vi "AD9910.vi"() -> ()   [LabVIEW 2018]
panel:
  in  "Name":string
  out "SN":u16 format="%04x"
  in  "Save Button":bool
  out "Save Config":path
  in  "Open Config":path
  out "Error":errorcluster
  in  "Stop":bool
  in  "Enable Sine Out":bool
  in  "Enable Profile ASF":bool
  in  "Profiles":enum32{"Single Tone", "RAM"}(tab)
  in  "Single Tone 0":T1 {"Phase" step=0.1 format="%.5f"; "Power" min=0.0 max=0.0009998779334127903 step=5e-05 format="%.9f"; "Frequency" min=0.0 max=500000000.0 format="%.7f"}
  in  "Single Tone 1":T1 {"Phase" step=0.1 format="%.5f"; "Power" min=0.0 max=0.0009998779334127903 step=5e-05 format="%.9f"; "Frequency" min=0.0 max=500000000.0 format="%.7f"}
  in  "Single Tone 2":T1 {"Phase" step=0.1 format="%.5f"; "Power" min=0.0 max=0.0009998779334127903 step=5e-05 format="%.9f"; "Frequency" min=0.0 max=500000000.0 format="%.7f"}
  in  "Single Tone 3":T1 {"Phase" step=0.1 format="%.5f"; "Power" min=0.0 max=0.0009998779334127903 step=5e-05 format="%.9f"; "Frequency" min=0.0 max=500000000.0 format="%.7f"}
  in  "Single Tone 4":T1 {"Phase" step=0.1 format="%.5f"; "Power" min=0.0 max=0.0009998779334127903 step=5e-05 format="%.9f"; "Frequency" min=0.0 max=500000000.0 format="%.7f"}
  in  "Single Tone 5":T1 {"Phase" step=0.1 format="%.5f"; "Power" min=0.0 max=0.0009998779334127903 step=5e-05 format="%.9f"; "Frequency" min=0.0 max=500000000.0 format="%.7f"}
  in  "Single Tone 6":T1 {"Phase" step=0.1 format="%.5f"; "Power" min=0.0 max=0.0009998779334127903 step=5e-05 format="%.9f"; "Frequency" min=0.0 max=500000000.0 format="%.7f"}
  in  "Single Tone 7":T1 {"Phase" step=0.1 format="%.5f"; "Power" min=0.0 max=0.0009998779334127903 step=5e-05 format="%.9f"; "Frequency" min=0.0 max=500000000.0 format="%.7f"}
  in  "Activate":T2(radio)
  in  "ADIClockEval":u16(ring) items=["not 780 X- Local Detection_is raman S&H", "780_X+_Local_Detection", "1529 Shielding", "420 S&H", "808 SLM", "420 Slow Feedback"]
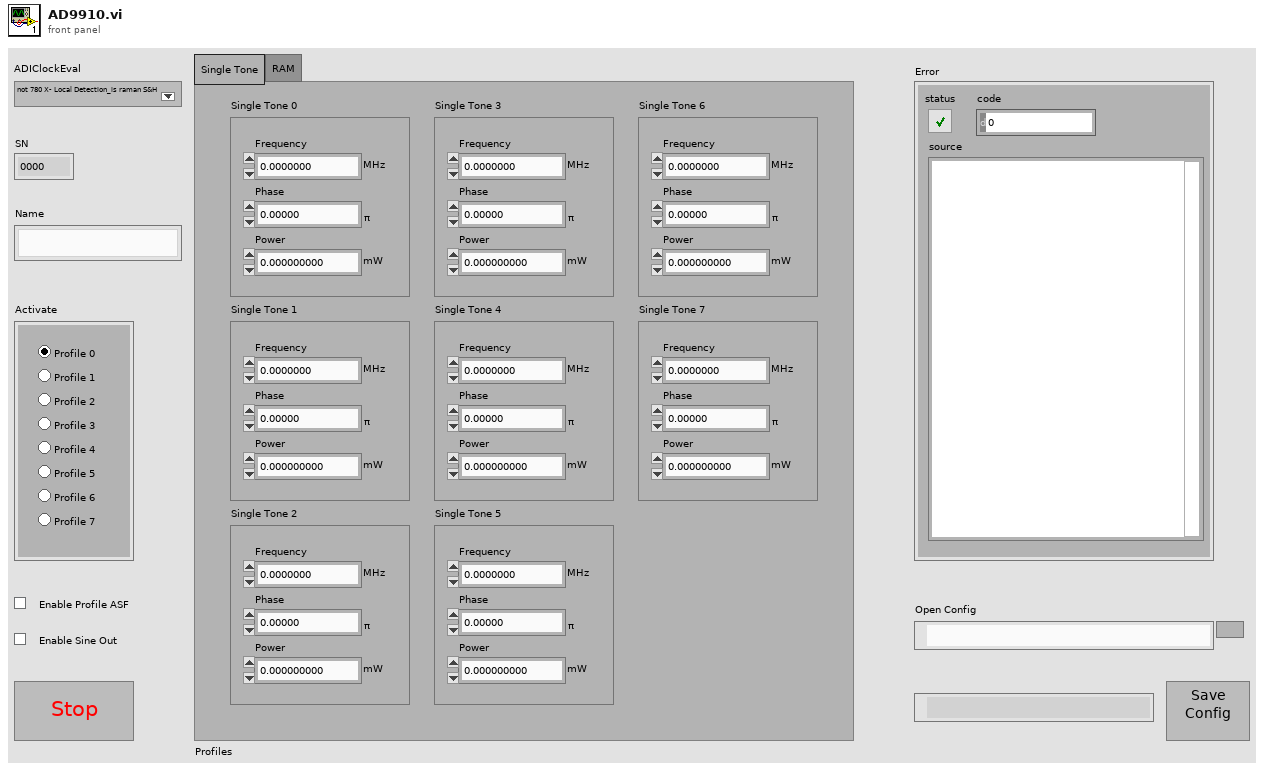
[diagram p1: front panel]
types:
  T1 = cluster{"Frequency":dbl[unit], "Phase":dbl, "Power":dbl[unit]}
  T2 = enum32{"单选选项0", "单选选项1", "单选选项2", "单选选项3", "单选选项4", "单选选项5", "单选选项6", "单选选项7"}
  T3 = cluster{"[0]":enum8{"Enabled", "Disabled", "Disabled and Grayed Out"}, "[1]":enum8{"Enabled", "Disabled", "Disabled and Grayed Out"}, "[2]":enum8{"Enabled", "Disabled", "Disabled and Grayed Out"}, "[3]":enum8{"Enabled", "Disabled", "Disabled and Grayed Out"}, "[4]":enum8{"Enabled", "Disabled", "Disabled and Grayed Out"}, "[5]":enum8{"Enabled", "Disabled", "Disabled and Grayed Out"}, "[6]":enum8{"Enabled", "Disabled", "Disabled and Grayed Out"}, "[7]":enum8{"Enabled", "Disabled", "Disabled and Grayed Out"}}
  T4 = cluster{"Single Tone 0":cluster{"Frequency":dbl[unit], "Phase":dbl, "Power":dbl[unit]}, "Single Tone 1":cluster{"Frequency":dbl[unit], "Phase":dbl, "Power":dbl[unit]}, "Single Tone 2":cluster{"Frequency":dbl[unit], "Phase":dbl, "Power":dbl[unit]}, "Single Tone 3":cluster{"Frequency":dbl[unit], "Phase":dbl, "Power":dbl[unit]}, "Single Tone 4":cluster{"Frequency":dbl[unit], "Phase":dbl, "Power":dbl[unit]}, "Single Tone 5":cluster{"Frequency":dbl[unit], "Phase":dbl, "Power":dbl[unit]}, "Single Tone 6":cluster{"Frequency":dbl[unit], "Phase":dbl, "Power":dbl[unit]}, "Single Tone 7":cluster{"Frequency":dbl[unit], "Phase":dbl, "Power":dbl[unit]}}
  T5 = enum8{"Enabled", "Disabled", "Disabled and Grayed Out"}
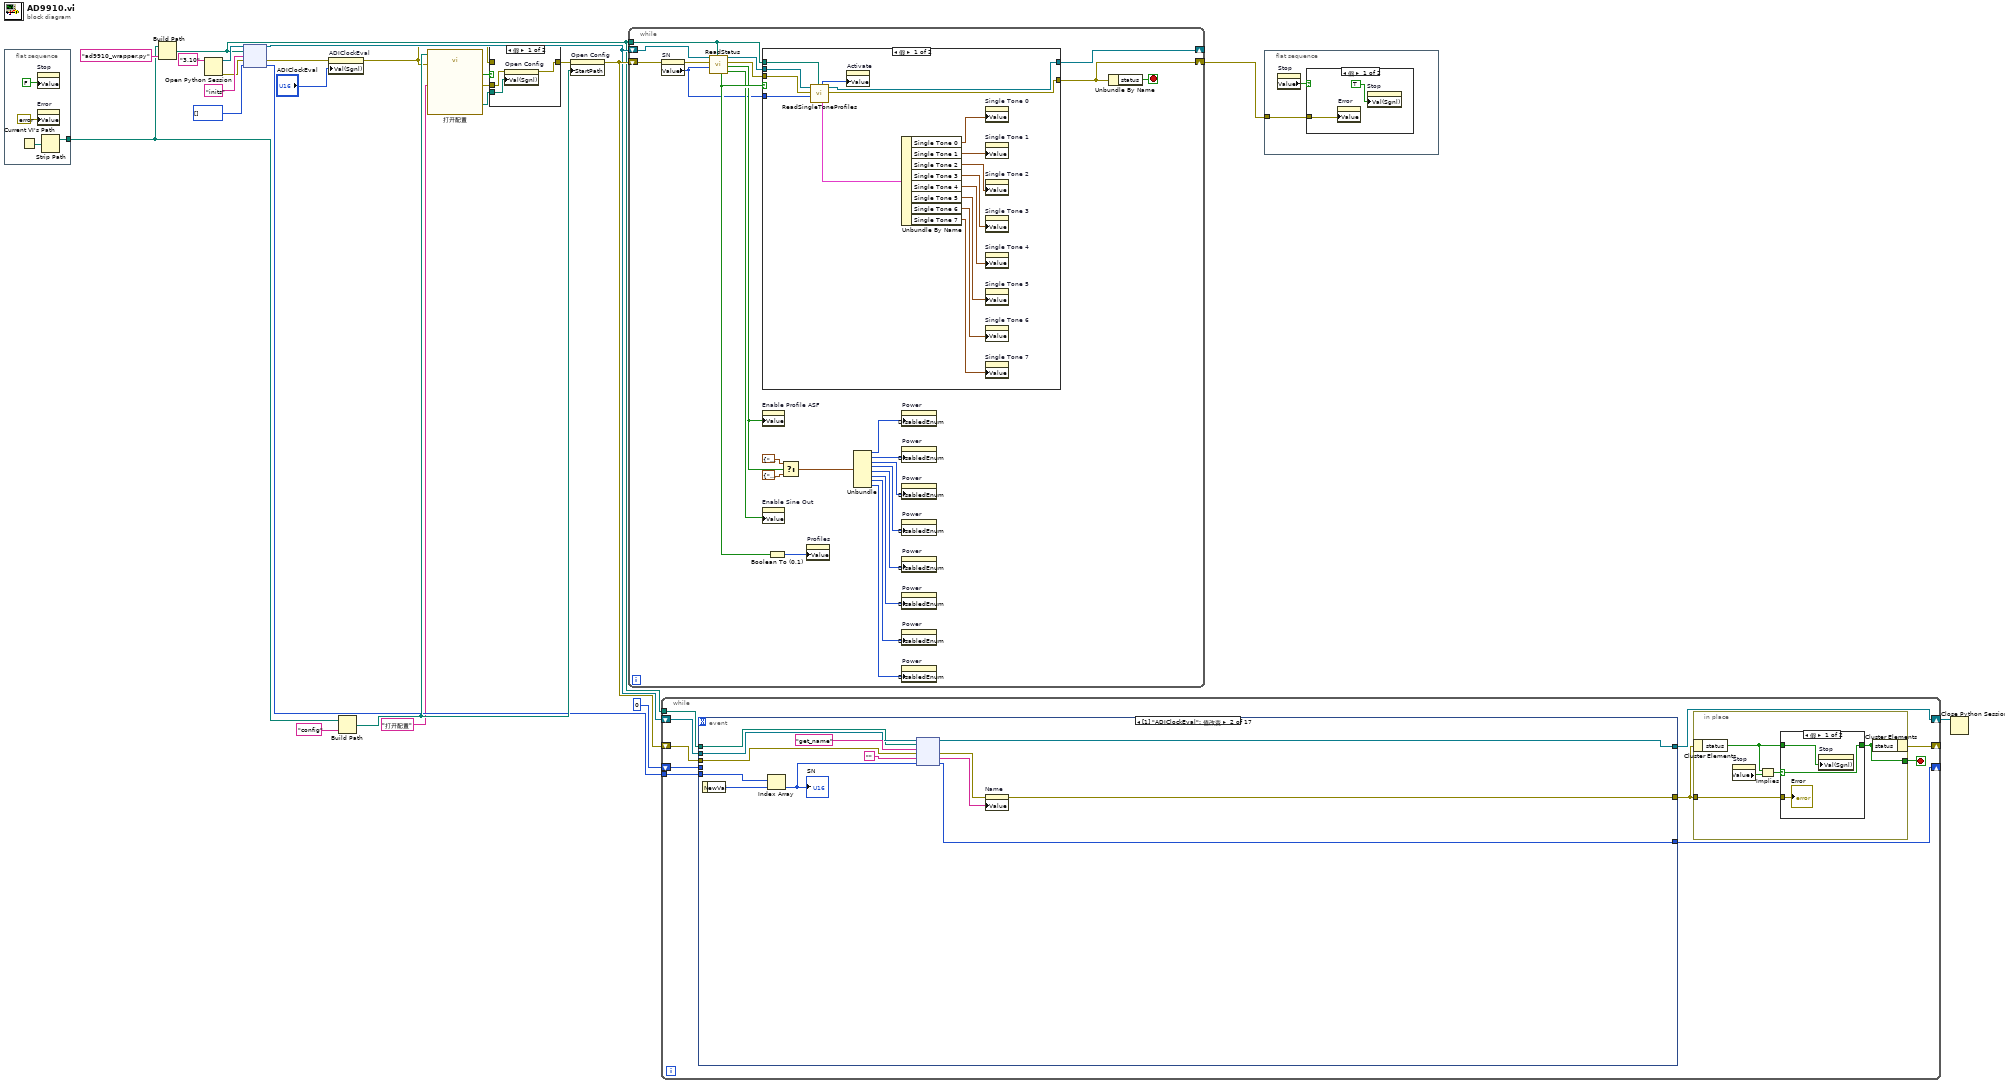
[diagram p0: block diagram]
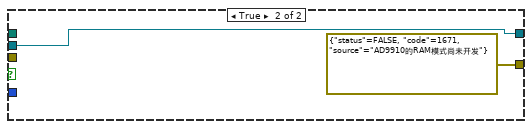
[diagram p4: hidden frame]
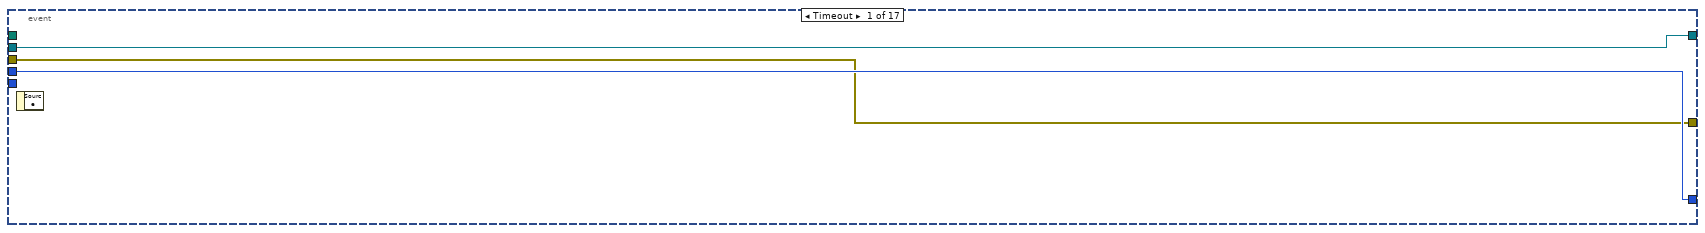
[diagram p6: hidden frame]
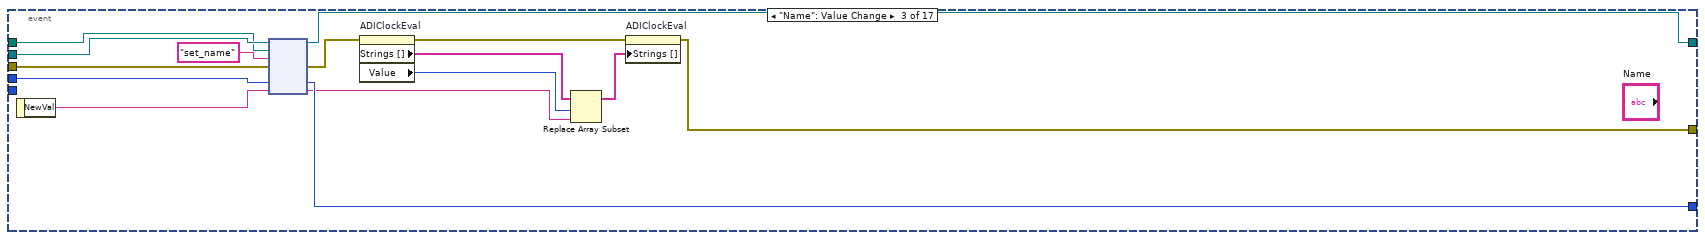
[diagram p7: hidden frame]
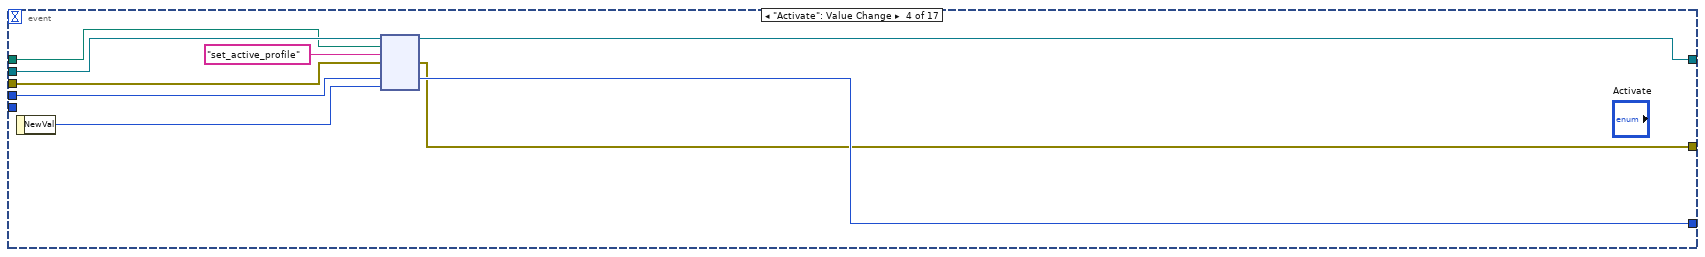
[diagram p8: hidden frame]
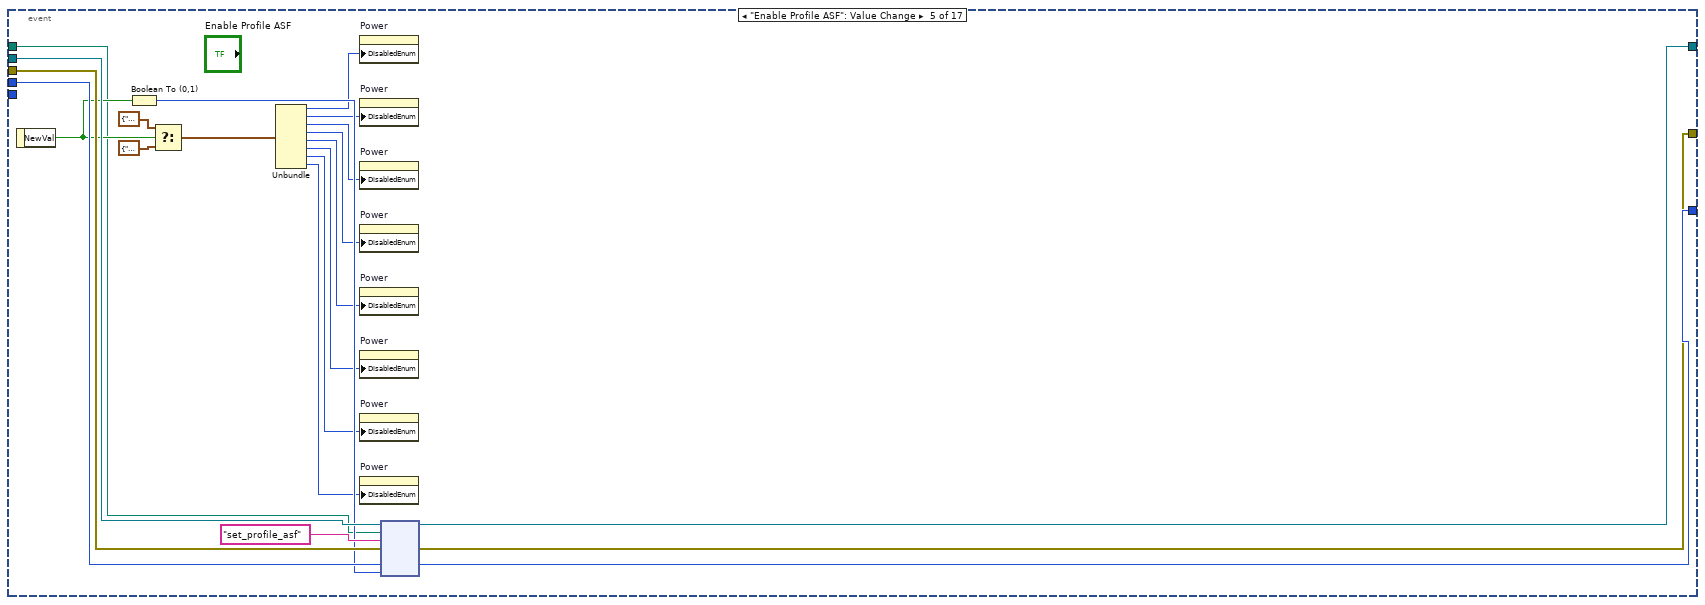
[diagram p9: hidden frame]
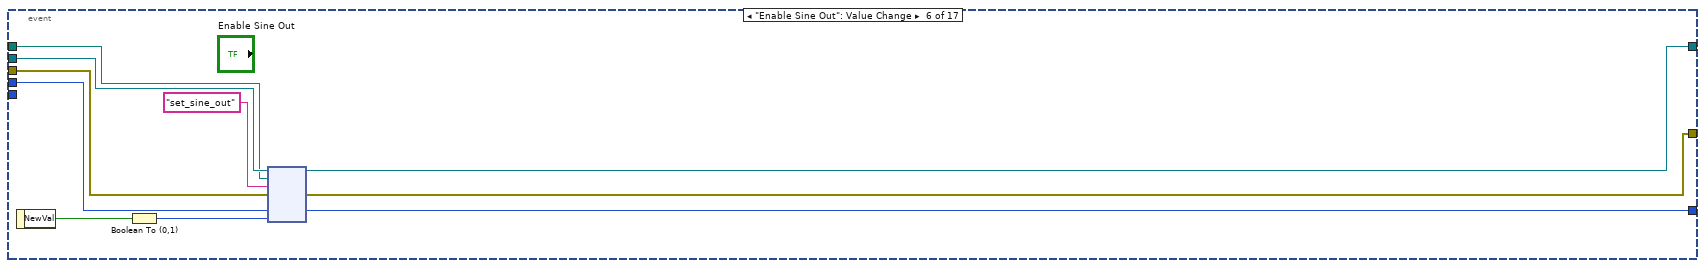
[diagram p10: hidden frame]
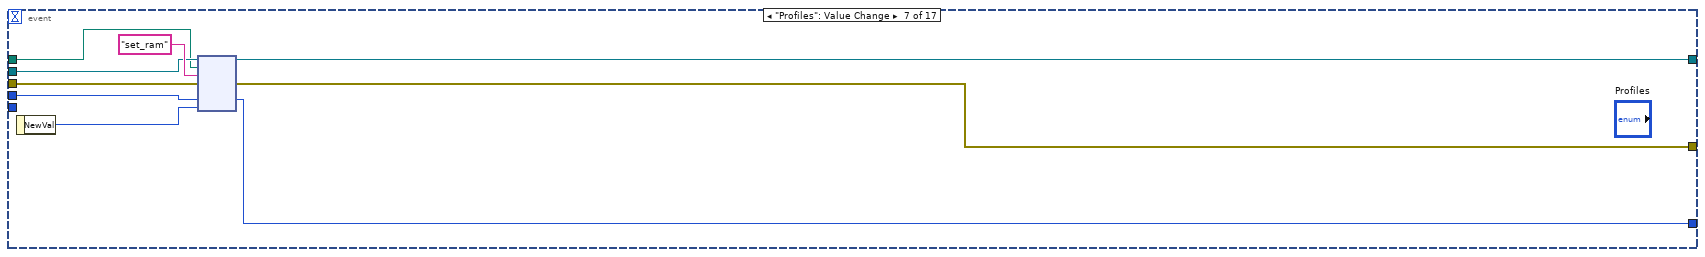
[diagram p11: hidden frame]
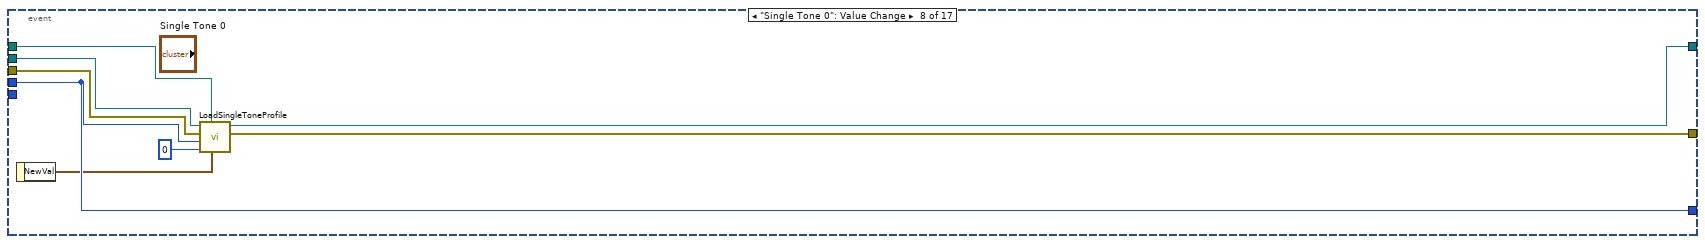
[diagram p12: hidden frame]
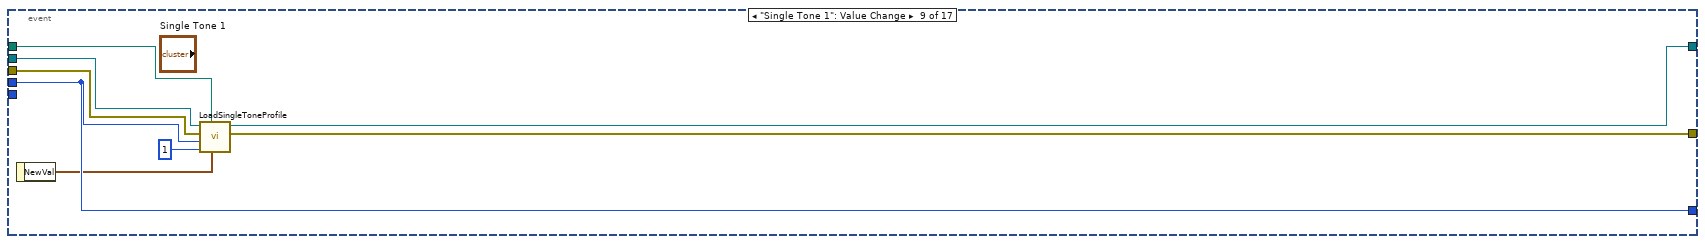
[diagram p13: hidden frame]
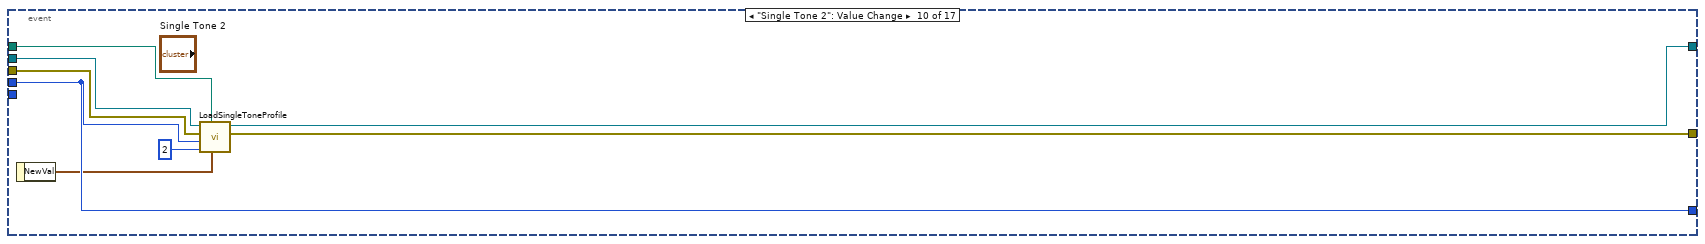
[diagram p14: hidden frame]
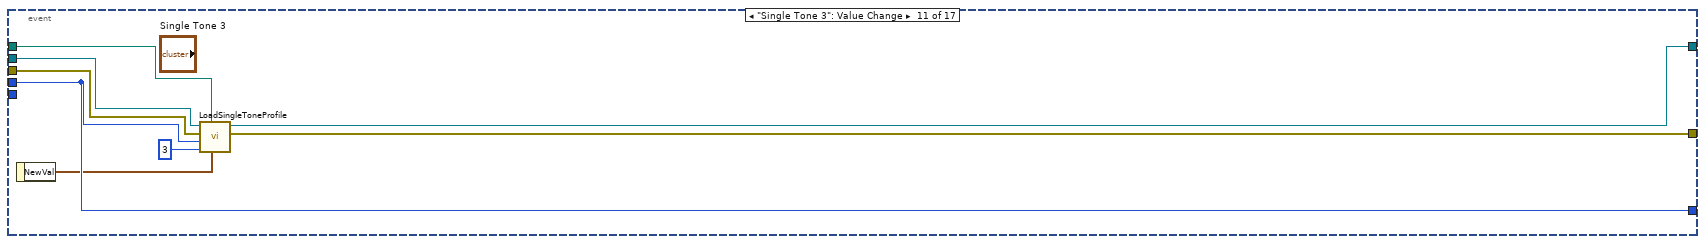
[diagram p15: hidden frame]
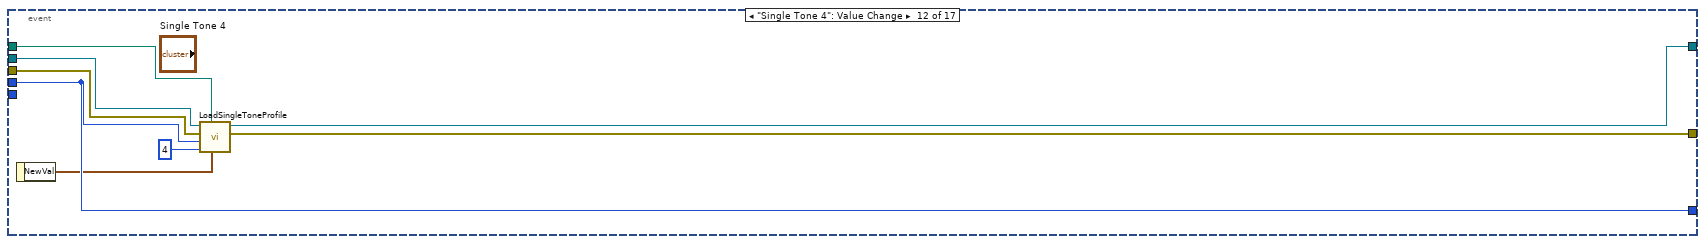
[diagram p16: hidden frame]
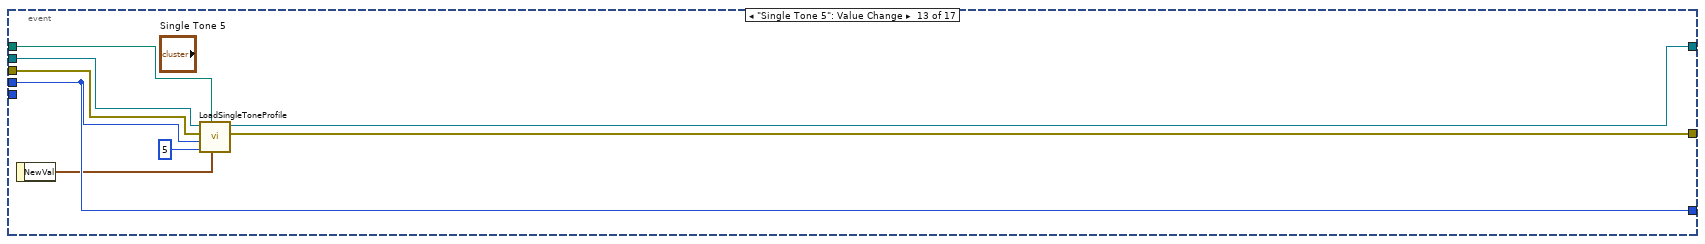
[diagram p17: hidden frame]
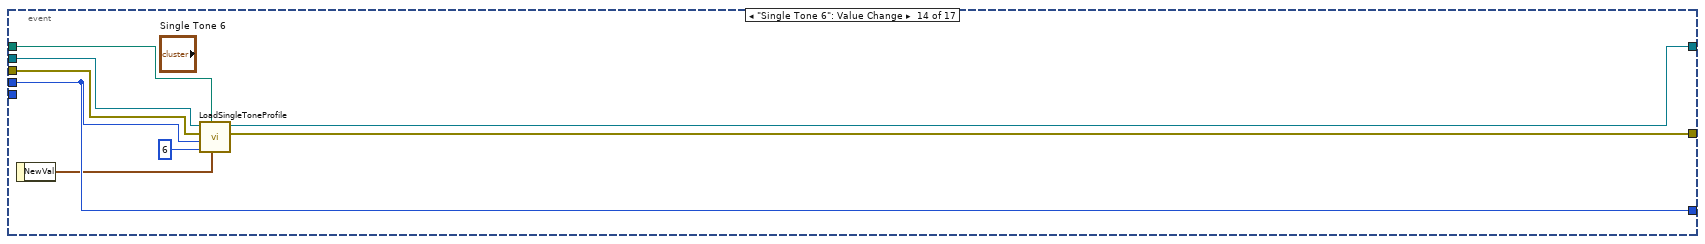
[diagram p18: hidden frame]
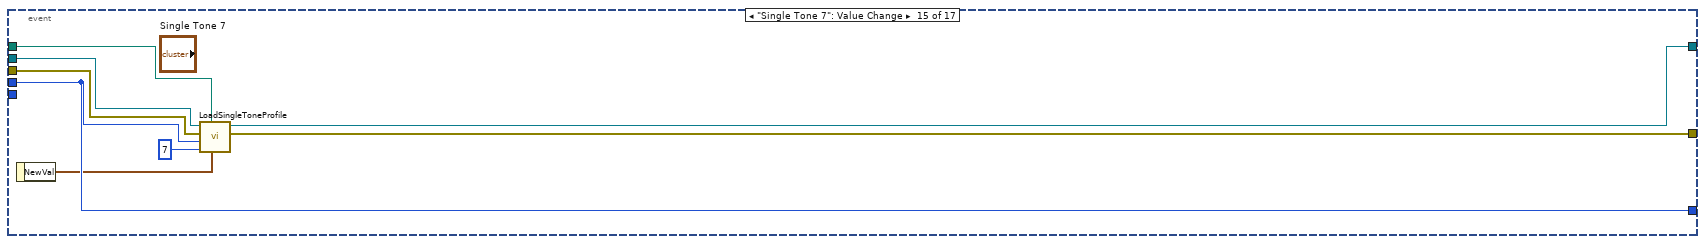
[diagram p19: hidden frame]
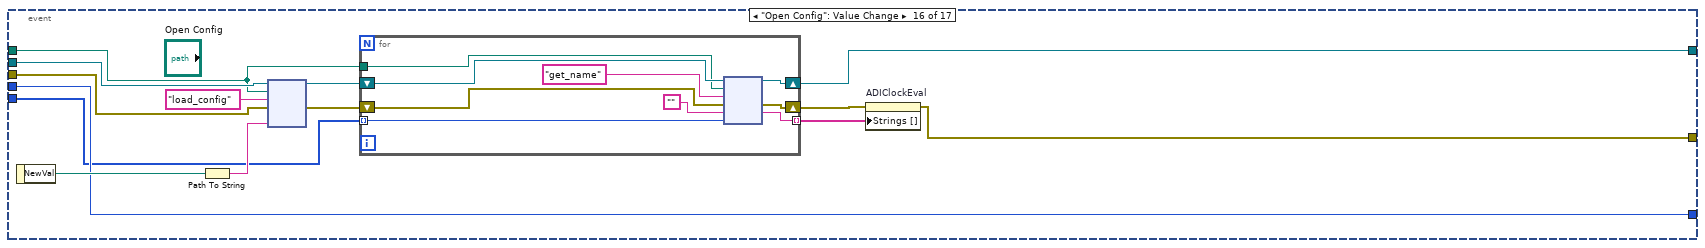
[diagram p20: hidden frame]
diagram:
  n1 = flat-sequence {
    tunnel: [w27] -> w16
    frame #0 {
      n2 = Current VI's Path() -> (path=w28:path)
      n3 = property on="Stop" class="Bool (严格)"("Value"=FALSE ("Stop")) -> ()  [unwired: 2 in, 2 out]
      n4 = property on="Error" class="Clust (严格)"("Value"=errorcluster {"status"=FALSE, "code"=0, "source"=""} ("Error")) -> ()  [unwired: 2 in, 2 out]
      n5 = Strip Path(path=w28) -> (stripped path=w27:path)  [unwired: 1 out]
    }
  }
  n6 = Build Path(base path=w16, name or relative path="ad9910_wrapper.py") -> (appended path=w10:path)
  n7 = Open Python Session(python version="3.10" ("Python版本")) -> (session out=w23:refnum<k35>, error out=w21:errorcluster)  [unwired: 2 in]
  n8 = node ("Python节点")(w23, w10, "inits", w21, u16[] []) -> (w11:refnum<k35>, w3:errorcluster, w9:u16[])  [unwired: 2 out]
  n9 = property on="ADIClockEval" class="Ring (严格)"(error in=w3, "Val(Sgnl)"="ADIClockEval") -> (error out=w2:errorcluster)  [unwired: 1 in, 1 out]
  n10 = Build Path(base path=w16, name or relative path="config") -> (appended path=w15:path)
  n11 = call "打开配置"("start path"=w15, "prompt"="打开配置" ("default name"), "error in"=w2) -> ("selected path"=w6:path, "cancelled"=w7:bool, "error out"=w5:errorcluster)  [unwired: 9 in, 1 out]
  n12 = case shown="假" w7 {
    tunnel: w6 -> [w31 _]
    tunnel: w5 -> [w30 _]
    tunnel: [w29 w32] -> w14
    tunnel: w2 -> [_ w32]
    frame False {
      n13 = property on="Open Config" class="Path"(error in=w30, "Val(Sgnl)"=w31) -> (error out=w29:errorcluster)  [unwired: 1 in, 1 out]
    }
    frame True {
    }
  }
  n14 = property on="Open Config" class="Path"(error in=w14, "StartPath"=w15) -> (error out=w13:errorcluster)  [unwired: 1 in, 1 out]
  n15 = while {
    shift-right: [w36] -> _
    shift-left: w11 -> [w42]
    shift-right: [w37] -> w18
    shift-left: w13 -> [w35]
    tunnel: w10 -> [w40]
    stop <- w41 stop-if-true
    n16 = property on="SN" class="DigNum (严格)"(error in=w35) -> (error out=w34:errorcluster, "Value"=w33:u16)  [unwired: 1 in, 1 out]
    n17 = call "ReadStatus.vi"("模块路径"=w40, "sn"=w33, "错误输入（无错误）"=w34, "会话句柄输入"=w42) -> ("Enable Sine Out"=w47:bool, "Enable Profile ASF"=w45:bool, "错误输出"=w39:errorcluster, "会话句柄输出"=w38:refnum<k35>, "Enable RAM"=w49:bool)  [unwired: 3 in]
    n18 = case shown="假" w49 {
      tunnel: w38 -> [w73 w74]
      tunnel: w39 -> [w72 _]
      tunnel: w33 -> [w71 _]
      tunnel: [w70 errorcluster {"status"=FALSE, "code"=1671, "source"="AD9910的RAM模式尚未开发"} ("错误输出")] -> w37
      tunnel: [w69 w74] -> w36
      tunnel: w40 -> [w58 _]
      frame False {
        n19 = call "ReadSingleToneProfiles.vi"("模块路径"=w58, "sn"=w71, "错误输入（无错误）"=w72, "会话句柄输入"=w73) -> ("错误输出"=w70:errorcluster, "会话句柄输出"=w69:refnum<k35>, "Single Tone Profiles"=w68:T4, "Activate"=w67:T2)  [unwired: 4 in]
        n20 = property on="Activate" class="RadioBtnsControl (严格)"("Value"=w67) -> ()  [unwired: 2 in, 2 out]
        n21 = Unbundle By Name(w68) -> ("Single Tone 0"=w66:T1, "Single Tone 1"=w65:T1, "Single Tone 2"=w64:T1, "Single Tone 3"=w63:T1, "Single Tone 4"=w62:T1, "Single Tone 5"=w61:T1, "Single Tone 6"=w60:T1, "Single Tone 7"=w59:T1)
        n22 = property on="Single Tone 0" class="Clust (严格)"("Value"=w66) -> ()  [unwired: 2 in, 2 out]
        n23 = property on="Single Tone 1" class="Clust (严格)"("Value"=w65) -> ()  [unwired: 2 in, 2 out]
        n24 = property on="Single Tone 2" class="Clust (严格)"("Value"=w64) -> ()  [unwired: 2 in, 2 out]
        n25 = property on="Single Tone 3" class="Clust (严格)"("Value"=w63) -> ()  [unwired: 2 in, 2 out]
        n26 = property on="Single Tone 4" class="Clust (严格)"("Value"=w62) -> ()  [unwired: 2 in, 2 out]
        n27 = property on="Single Tone 5" class="Clust (严格)"("Value"=w61) -> ()  [unwired: 2 in, 2 out]
        n28 = property on="Single Tone 6" class="Clust (严格)"("Value"=w60) -> ()  [unwired: 2 in, 2 out]
        n29 = property on="Single Tone 7" class="Clust (严格)"("Value"=w59) -> ()  [unwired: 2 in, 2 out]
      }
      frame True {
      }
    }
    n30 = property on="Enable Profile ASF" class="Bool (严格)"("Value"=w45) -> ()  [unwired: 2 in, 2 out]
    n31 = property on="Enable Sine Out" class="Bool (严格)"("Value"=w47) -> ()  [unwired: 2 in, 2 out]
    n32 = Boolean To (0,1)(Boolean=w49) -> (0, 1=w48:i16)
    n33 = Select(t=T3 {"[0]"=enum."Enabled", "[1]"=enum."Enabled", "[2]"=enum."Enabled", "[3]"=enum."Enabled", "[4]"=enum."Enabled", "[5]"=enum."Enabled", "[6]"=enum."Enabled", "[7]"=enum."Enabled"} ("簇"), s=w45, f=T3 {"[0]"=enum."Disabled and Grayed Out", "[1]"=enum."Disabled and Grayed Out", "[2]"=enum."Disabled and Grayed Out", "[3]"=enum."Disabled and Grayed Out", "[4]"=enum."Disabled and Grayed Out", "[5]"=enum."Disabled and Grayed Out", "[6]"=enum."Disabled and Grayed Out", "[7]"=enum."Disabled and Grayed Out"} ("簇")) -> (s? t:f=w46:T3)
    n34 = property on="Profiles" class="TabCtl (严格)"("Value"=w48) -> ()  [unwired: 2 in, 2 out]
    n35 = Unbundle(w46) -> ("[0]"=w50:T5, "[1]"=w51:T5, "[2]"=w52:T5, "[3]"=w53:T5, "[4]"=w54:T5, "[5]"=w55:T5, "[6]"=w56:T5, "[7]"=w57:T5)
    n36 = property on="Power" class="DigNum (严格)"("DisabledEnum"=w50) -> ()  [unwired: 2 in, 2 out]
    n37 = property on="Power" class="DigNum (严格)"("DisabledEnum"=w51) -> ()  [unwired: 2 in, 2 out]
    n38 = property on="Power" class="DigNum (严格)"("DisabledEnum"=w52) -> ()  [unwired: 2 in, 2 out]
    n39 = property on="Power" class="DigNum (严格)"("DisabledEnum"=w53) -> ()  [unwired: 2 in, 2 out]
    n40 = property on="Power" class="DigNum (严格)"("DisabledEnum"=w54) -> ()  [unwired: 2 in, 2 out]
    n41 = property on="Power" class="DigNum (严格)"("DisabledEnum"=w55) -> ()  [unwired: 2 in, 2 out]
    n42 = property on="Power" class="DigNum (严格)"("DisabledEnum"=w56) -> ()  [unwired: 2 in, 2 out]
    n43 = property on="Power" class="DigNum (严格)"("DisabledEnum"=w57) -> ()  [unwired: 2 in, 2 out]
    n44 = Unbundle By Name(w37) -> ("status"=w41:bool)
  }
  n45 = while {
    tunnel: w9 -> [w80]
    shift-right: [w82] -> _
    shift-left: u16 0 -> [w84]
    shift-right: [w78] -> _
    shift-left: w13 -> [w81]
    shift-right: [w83] -> w12
    shift-left: w11 -> [w85]
    tunnel: w10 -> [w79]
    stop <- w77 stop-if-true
    n46 = event shown="[1] \"ADIClockEval\": 值改变" {
      selector: _ -> [_ _ _ _ _ _ _ _ _ _ _ _ _ _ _ _ _]
      dyn-events: _ -> [_ _ _ _ _ _ _ _ _ _ _ _ _ _ _ _ _]
      timeout: _ -> [_ _ _ _ _ _ _ _ _ _ _ _ _ _ _ _ _]
      tunnel: w81 -> [w96 w98 w122 w133 w153 w163 w172 w181 w189 w197 w205 w213 w221 w229 w237 w248 w284]
      tunnel: w85 -> [w95 w104 w125 w134 w154 w164 w173 w182 w190 w198 w206 w214 w222 w230 w238 w249 w274]
      tunnel: w84 -> [w97 _ w121 w132 w152 w162 w171 w178 w186 w194 w202 w210 w218 w226 w234 w247 w268]
      tunnel: [w95 w103 w119 w129 w149 w158 w170 w177 w185 w193 w201 w209 w217 w225 w233 w243 w263] -> w83
      tunnel: [w97 w102 w118 w130 w150 w160 w168 w178 w186 w194 w202 w210 w218 w226 w234 w247 w268] -> w82
      tunnel: w80 -> [_ w109 _ _ _ _ _ _ _ _ _ _ _ _ _ w246 _]
      tunnel: w79 -> [_ w101 w124 w126 w135 w156 w166 w175 w183 w191 w199 w207 w215 w223 w231 w242 w262]
      tunnel: [w96 w100 w113 w128 w148 w159 w169 w179 w187 w195 w203 w211 w219 w227 w235 w240 w265] -> w76
      event Timeout {
        n47 = event-data() -> ()  [unwired: 1 in, 1 out]
      }
      event "ADIClockEval": Value Change {
        n48 = event-data() -> ("NewVal"=w110:u16)  [unwired: 1 in]
        n49 = Index Array(array=w109, index=w110) -> (element=w99:u16)
        "SN" <- w99
        n50 = node(w104, w101, "get_name", w98, "", w99) -> (w103:refnum<k35>, w108:errorcluster, w107:string, w102:u16)  [unwired: 2 out]
        n51 = property on="Name" class="Str"(error in=w108, "Value"=w107) -> (error out=w100:errorcluster)  [unwired: 1 in, 1 out]
      }
      event "Name": Value Change {
        n52 = event-data() -> ("NewVal"=w120:string)  [unwired: 1 in]
        n53 = node(w125, w124, "set_name", w122, w121, w120) -> (w119:refnum<k35>, w117:errorcluster, w118:u16, w114:string)  [unwired: 2 in, 2 out]
        n54 = property on="ADIClockEval" class="Ring (严格)"(error in=w117) -> (error out=w111:errorcluster, "Strings []"=w116:string[], "Value"=w115:u16)  [unwired: 1 in, 1 out]
        n55 = Replace Array Subset(array=w116, new element=w114, index=w115) -> (w112:string[])
        n56 = property on="ADIClockEval" class="Ring (严格)"(error in=w111, "Strings []"=w112) -> (error out=w113:errorcluster)  [unwired: 1 in, 1 out]
      }
      event "Activate": Value Change {
        n57 = event-data() -> ("NewVal"=w127:T2)  [unwired: 1 in]
        n58 = node(w134, w126, "set_active_profile", w133, w132, w127) -> (w129:refnum<k35>, w128:errorcluster, w130:u16)  [unwired: 3 in, 2 out]
      }
      event "Enable Profile ASF": Value Change {
        n59 = event-data() -> ("NewVal"=w136:bool)  [unwired: 1 in]
        n60 = Boolean To (0,1)(Boolean=w136) -> (0, 1=w151:i16)
        n61 = Select(t=T3 {"[0]"=enum."Enabled", "[1]"=enum."Enabled", "[2]"=enum."Enabled", "[3]"=enum."Enabled", "[4]"=enum."Enabled", "[5]"=enum."Enabled", "[6]"=enum."Enabled", "[7]"=enum."Enabled"} ("簇"), s=w136, f=T3 {"[0]"=enum."Disabled and Grayed Out", "[1]"=enum."Disabled and Grayed Out", "[2]"=enum."Disabled and Grayed Out", "[3]"=enum."Disabled and Grayed Out", "[4]"=enum."Disabled and Grayed Out", "[5]"=enum."Disabled and Grayed Out", "[6]"=enum."Disabled and Grayed Out", "[7]"=enum."Disabled and Grayed Out"} ("簇")) -> (s? t:f=w147:T3)
        n62 = Unbundle(w147) -> ("[0]"=w146:T5, "[1]"=w145:T5, "[2]"=w144:T5, "[3]"=w143:T5, "[4]"=w142:T5, "[5]"=w141:T5, "[6]"=w140:T5, "[7]"=w139:T5)
        n63 = property on="Power" class="DigNum (严格)"("DisabledEnum"=w146) -> ()  [unwired: 2 in, 2 out]
        n64 = property on="Power" class="DigNum (严格)"("DisabledEnum"=w145) -> ()  [unwired: 2 in, 2 out]
        n65 = property on="Power" class="DigNum (严格)"("DisabledEnum"=w144) -> ()  [unwired: 2 in, 2 out]
        n66 = property on="Power" class="DigNum (严格)"("DisabledEnum"=w143) -> ()  [unwired: 2 in, 2 out]
        n67 = property on="Power" class="DigNum (严格)"("DisabledEnum"=w142) -> ()  [unwired: 2 in, 2 out]
        n68 = property on="Power" class="DigNum (严格)"("DisabledEnum"=w141) -> ()  [unwired: 2 in, 2 out]
        n69 = property on="Power" class="DigNum (严格)"("DisabledEnum"=w140) -> ()  [unwired: 2 in, 2 out]
        n70 = property on="Power" class="DigNum (严格)"("DisabledEnum"=w139) -> ()  [unwired: 2 in, 2 out]
        n71 = node(w154, w135, "set_profile_asf", w153, w152, w151) -> (w149:refnum<k35>, w148:errorcluster, w150:u16)  [unwired: 3 in, 2 out]
      }
      event "Enable Sine Out": Value Change {
        n72 = event-data() -> ("NewVal"=w157:bool)  [unwired: 1 in]
        n73 = Boolean To (0,1)(Boolean=w157) -> (0, 1=w161:i16)
        n74 = node(w164, w156, "set_sine_out", w163, w162, w161) -> (w158:refnum<k35>, w159:errorcluster, w160:u16)  [unwired: 3 in, 2 out]
      }
      event "Profiles": Value Change {
        n75 = event-data() -> ("NewVal"=w167:enum32{"Single Tone", "RAM"})  [unwired: 1 in]
        n76 = node(w173, w166, "set_ram", w172, w171, w167) -> (w170:refnum<k35>, w169:errorcluster, w168:u16)  [unwired: 3 in, 2 out]
      }
      event "Single Tone 0": Value Change {
        n77 = event-data() -> ("NewVal"=w176:T1)  [unwired: 1 in]
        n78 = call "LoadSingleToneProfile.vi"("Single Tone"=w176, "模块路径"=w175, "PF"=u8 0, "sn"=w178, "错误输入（无错误）"=w181, "会话句柄输入"=w182) -> ("错误输出"=w179:errorcluster, "会话句柄输出"=w177:refnum<k35>)  [unwired: 4 in]
      }
      event "Single Tone 1": Value Change {
        n79 = event-data() -> ("NewVal"=w184:T1)  [unwired: 1 in]
        n80 = call "LoadSingleToneProfile.vi"("Single Tone"=w184, "模块路径"=w183, "PF"=u8 1, "sn"=w186, "错误输入（无错误）"=w189, "会话句柄输入"=w190) -> ("错误输出"=w187:errorcluster, "会话句柄输出"=w185:refnum<k35>)  [unwired: 4 in]
      }
      event "Single Tone 2": Value Change {
        n81 = event-data() -> ("NewVal"=w192:T1)  [unwired: 1 in]
        n82 = call "LoadSingleToneProfile.vi"("Single Tone"=w192, "模块路径"=w191, "PF"=u8 2, "sn"=w194, "错误输入（无错误）"=w197, "会话句柄输入"=w198) -> ("错误输出"=w195:errorcluster, "会话句柄输出"=w193:refnum<k35>)  [unwired: 4 in]
      }
      event "Single Tone 3": Value Change {
        n83 = event-data() -> ("NewVal"=w200:T1)  [unwired: 1 in]
        n84 = call "LoadSingleToneProfile.vi"("Single Tone"=w200, "模块路径"=w199, "PF"=u8 3, "sn"=w202, "错误输入（无错误）"=w205, "会话句柄输入"=w206) -> ("错误输出"=w203:errorcluster, "会话句柄输出"=w201:refnum<k35>)  [unwired: 4 in]
      }
      event "Single Tone 4": Value Change {
        n85 = event-data() -> ("NewVal"=w208:T1)  [unwired: 1 in]
        n86 = call "LoadSingleToneProfile.vi"("Single Tone"=w208, "模块路径"=w207, "PF"=u8 4, "sn"=w210, "错误输入（无错误）"=w213, "会话句柄输入"=w214) -> ("错误输出"=w211:errorcluster, "会话句柄输出"=w209:refnum<k35>)  [unwired: 4 in]
      }
      event "Single Tone 5": Value Change {
        n87 = event-data() -> ("NewVal"=w216:T1)  [unwired: 1 in]
        n88 = call "LoadSingleToneProfile.vi"("Single Tone"=w216, "模块路径"=w215, "PF"=u8 5, "sn"=w218, "错误输入（无错误）"=w221, "会话句柄输入"=w222) -> ("错误输出"=w219:errorcluster, "会话句柄输出"=w217:refnum<k35>)  [unwired: 4 in]
      }
      event "Single Tone 6": Value Change {
        n89 = event-data() -> ("NewVal"=w224:T1)  [unwired: 1 in]
        n90 = call "LoadSingleToneProfile.vi"("Single Tone"=w224, "模块路径"=w223, "PF"=u8 6, "sn"=w226, "错误输入（无错误）"=w229, "会话句柄输入"=w230) -> ("错误输出"=w227:errorcluster, "会话句柄输出"=w225:refnum<k35>)  [unwired: 4 in]
      }
      event "Single Tone 7": Value Change {
        n91 = event-data() -> ("NewVal"=w232:T1)  [unwired: 1 in]
        n92 = call "LoadSingleToneProfile.vi"("Single Tone"=w232, "模块路径"=w231, "PF"=u8 7, "sn"=w234, "错误输入（无错误）"=w237, "会话句柄输入"=w238) -> ("错误输出"=w235:errorcluster, "会话句柄输出"=w233:refnum<k35>)  [unwired: 4 in]
      }
      event "Open Config": Value Change {
        n93 = event-data() -> ("NewVal"=w252:path)  [unwired: 1 in]
        n94 = Path To String(path=w252) -> (string=w251:string)
        n95 = node(w249, w242, "load_config", w248, w251) -> (w244:refnum<k35>, w245:errorcluster)  [unwired: 3 in, 2 out]
        n96 = for {
          tunnel: w246 -> [w259] mode=indexing
          tunnel: [w258] -> w239 mode=indexing
          shift-right: [w256] -> w243
          shift-left: w244 -> [w257]
          tunnel: w242 -> [w255]
          shift-right: [w253] -> w241
          shift-left: w245 -> [w254]
          n97 = node(w257, w255, "get_name", w254, "", w259) -> (w256:refnum<k35>, w253:errorcluster, w258:string)  [unwired: 1 in, 2 out]
        }
        n98 = property on="ADIClockEval" class="Ring (严格)"(error in=w241, "Strings []"=w239) -> (error out=w240:errorcluster)  [unwired: 1 in, 1 out]
      }
      event "Save Button", "Stop": Value Change {
        n99 = event-data() -> ()  [unwired: 1 in, 1 out]
        n100 = property on="Save Button" class="Bool (严格)"(error in=w284, "Value"=FALSE ("Save Button")) -> (error out=w275:errorcluster)  [unwired: 1 in, 1 out]
        n101 = node(w274, w262, "get_path" ("function name"), w275, "") -> (w269:refnum<k35>, w271:errorcluster, w279:string)  [unwired: 2 out]
        n102 = String To Path(string=w279) -> (path=w278:path)
        n103 = Strip Path(path=w278) -> (stripped path=w276:path, name=w277:string)
        n104 = call "保存配置"("start path"=w276, "prompt"="保存配置", "default name"=w277, "error in"=w271) -> ("selected path"=w272:path, "cancelled"=w273:bool, "error out"=w270:errorcluster)  [unwired: 8 in, 1 out]
        n105 = case shown="假" w273 {
          tunnel: w272 -> [w302 _]
          tunnel: w271 -> [_ w306]
          tunnel: w270 -> [w303 _]
          tunnel: [w301 w306] -> w266
          tunnel: w269 -> [w300 w305]
          tunnel: [w299 w305] -> w264
          tunnel: w262 -> [w298 _]
          frame False {
            n106 = Path To String(path=w302) -> (string=w296:string)
            n107 = node(w300, w298, "save_config", w303, w296, w296) -> (w299:refnum<k35>, w301:errorcluster, w295:string)  [unwired: 1 in, 2 out]
            n108 = String To Path(string=w295) -> (path=→"Save Config":path)
          }
          frame True {
          }
        }
        n109 = case shown="真" "Stop" {
          tunnel: w266 -> [w286 w293]
          tunnel: [w286 w287] -> w265
          tunnel: w264 -> [w285 w292]
          tunnel: [w285 w291] -> w263
          tunnel: w262 -> [_ w290]
          frame False {
          }
          frame True {
            n110 = node(w292, w290, "deletes", w293) -> (w291:refnum<k35>, w289:errorcluster)  [unwired: 2 in, 2 out]
            n111 = Bundle By Name(cluster=w289, "status"=TRUE) -> (w287:errorcluster)
          }
        }
      }
    }
    n112 = in-place {
      in-place-border: [w90] -> w77
      in-place-border: w76 -> [w87]
      n113 = in-place-cluster #1(w76) -> ("status"=w88:bool)
      n114 = property on="Stop" class="Bool (严格)"() -> ("Value"=w86:bool)  [unwired: 2 in, 2 out]
      n115 = Implies(1:w86, 2:w88) -> (0:w89:bool)
      n116 = case shown="假" w89 {
        selector: w89 -> [w93 _]
        tunnel: [w93 w94] -> w90
        tunnel: w88 -> [w91 w94]
        tunnel: w87 -> [w92 _]
        frame False {
          n117 = property on="Stop" class="Bool (严格)"("Val(Sgnl)"=w91) -> ()  [unwired: 2 in, 2 out]
          "Error" <- w92
        }
        frame True {
        }
      }
      n118 = in-place-cluster #1("status"=w90) -> (w78:errorcluster)
    }
  }
  n119 = flat-sequence {
    tunnel: w18 -> [w308]
    frame #0 {
      n120 = property on="Stop" class="Bool (严格)"() -> ("Value"=w307:bool)  [unwired: 2 in, 2 out]
      n121 = case shown="假" w307 {
        tunnel: w308 -> [w309 _]
        frame False {
          n122 = property on="Error" class="Clust (严格)"("Value"=w309) -> ()  [unwired: 2 in, 2 out]
          n123 = property on="Stop" class="Bool (严格)"("Val(Sgnl)"=TRUE ("值(信号)")) -> ()  [unwired: 2 in, 2 out]
        }
        frame True {
        }
      }
    }
  }
  n124 = Close Python Session(session in=w12) -> ()  [unwired: 1 in, 1 out]
